vi "Lookup Channel.vi"(10 "channel":string, 11 "Channel Feedback":T1) -> (2 "found":bool, 3 "value":dbl)   [LabVIEW 2026]
doc: "Finds a channel by exact name in a Channel Feedback and returns its value. Linear search; an unknown channel answers found FALSE and value 0. Pure function, no error terminals, AF-free."
uses:
  Typedefs/Channel Value.ctl
  Typedefs/Channel Feedback.ctl
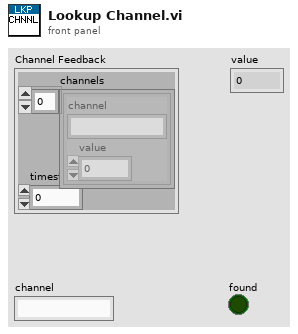
[diagram p1: front panel]
types:
  T1 = typedef "Channel Feedback.ctl" = cluster{"channels":T2[], "timestamp_ms":dbl}
  T2 = typedef "Channel Value.ctl" = cluster{"channel":string, "value":dbl}
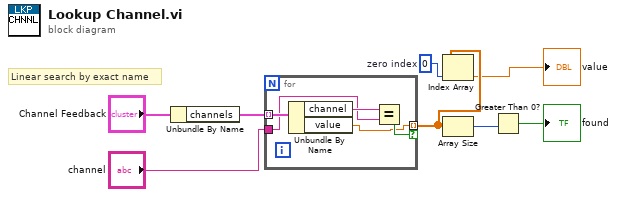
[diagram p0: block diagram]
diagram:
  w5 = 0  # zero index
  # "Linear search by exact name"
  n1 = Unbundle By Name("Channel Feedback") -> ("channels"=w7:T2[])
  n2 = for {
    tunnel: w7 -> [w13] mode=indexing
    tunnel: "channel" -> [w11]
    tunnel: [w9] -> w4 mode=indexing if=w10
    n3 = Unbundle By Name(w13) -> ("channel"=w12:string, "value"=w9:dbl)
    n4 = Equal?(x=w12, y=w11) -> (x = y?=w10:bool)
  }
  n5 = Index Array(array=w4, index=w5) -> (element=→"value":dbl)
  n6 = Array Size(array=w4) -> (size(s)=w3:i32)
  n7 = Greater Than 0?(x=w3) -> (x > 0?=→"found":bool)
